vi "set Limit Line Setting.vi"(8 "error in (no error)":errorcluster, 9 "Turn On?":bool, 10 "Limit Line Setting":T1={"Limit Line Index"=1, "Frequency Table"=[], "Amplitude Table"=[], "Name"=""} {"Limit Line Index" min=1 max=8}, 11 "Keysight 9020A in":refnum<class "Keysight 9020A.lvclass">) -> (0 "error out":errorcluster, 3 "Keysight 9020A out":refnum<class "Keysight 9020A.lvclass">)   [LabVIEW 2023, in "Spectrum Analyzer.lvlib" / "Keysight 9020A.lvclass"]
uses:
  Keysight 9020A.lvclass
  TYPE DEFINITION/TYPE Limit Line Setting Table.ctl
  Keysight 9020A.lvclass/Keysight 9020A.ctl
  Spectrum Analyzer.lvlib
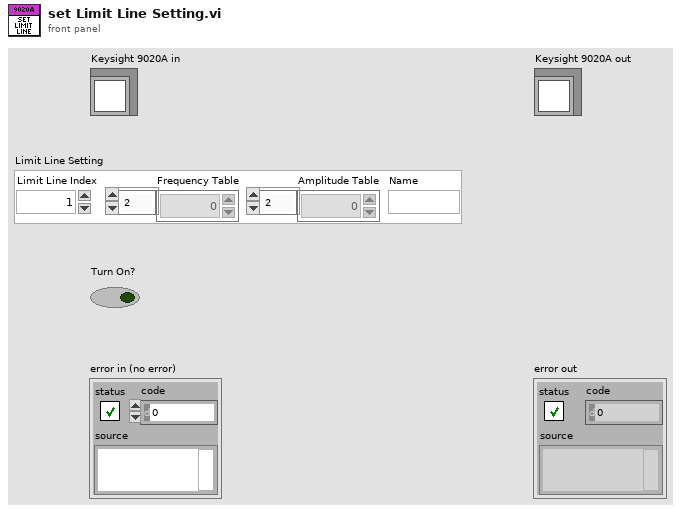
[diagram p1: front panel]
types:
  T1 = typedef "Spectrum Analyzer.lvlib/TYPE Limit Line Setting Table.ctl" = cluster{"Limit Line Index":i32, "Frequency Table":dbl[], "Amplitude Table":dbl[], "Name":string}
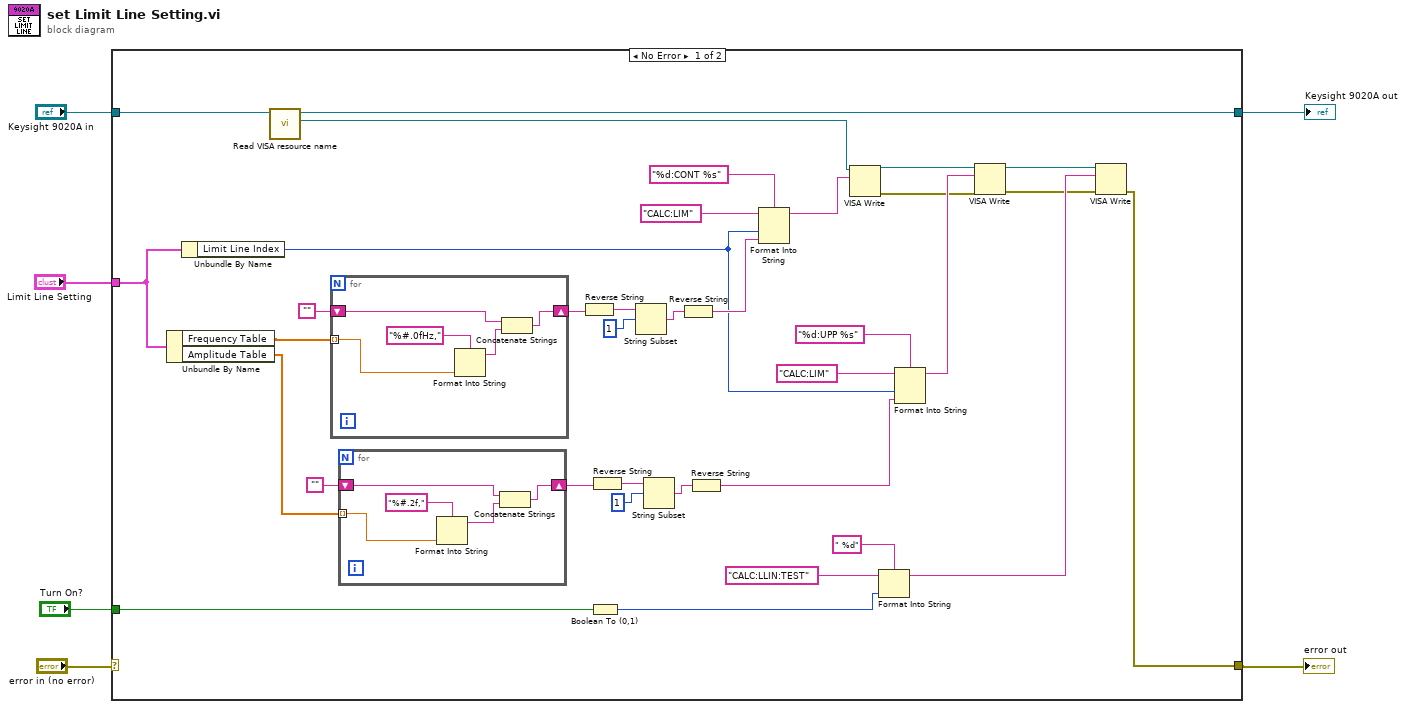
[diagram p0: block diagram]
diagram:
  n1 = case shown="No Error" "error in (no error)" {
    selector: "error in (no error)" -> [_ w52]
    tunnel: "Keysight 9020A in" -> [w40 w53]
    tunnel: [w41 w53] -> w5
    tunnel: [w8 w52] -> w3
    tunnel: "Limit Line Setting" -> [w33 _]
    tunnel: "Turn On?" -> [w15 _]
    frame No Error {
      n2 = Unbundle By Name(w33) -> ("Frequency Table"=w34:dbl[], "Amplitude Table"=w23:dbl[])
      n3 = Unbundle By Name(w33) -> ("Limit Line Index"=w20:i32)
      n4 = call "Read VISA resource name.vi"("Keysight 9020A in"=w40) -> ("VISA resource name"=w7:refnum<visa-resource-name>, "Keysight 9020A out"=w41:refnum<class "Keysight 9020A.lvclass">)  [unwired: 8 in, 1 out]
      n5 = for {
        tunnel: w34 -> [w47] mode=indexing
        shift-right: [w50] -> w38
        shift-left: "" -> [w51]
        n6 = Format Into String(format string="%#.0fHz,", w47) -> (resulting string=w48:string)  [unwired: 2 in, 1 out]
        n7 = Concatenate Strings(w51, w48) -> (w50:string)
      }
      n8 = for {
        tunnel: w23 -> [w44] mode=indexing
        shift-right: [w45] -> w25
        shift-left: "" -> [w46]
        n9 = Format Into String(format string="%#.2f,", w44) -> (resulting string=w43:string)  [unwired: 2 in, 1 out]
        n10 = Concatenate Strings(w46, w43) -> (w45:string)
      }
      n11 = Reverse String(1:w38) -> (0:w37:string)
      n12 = Boolean To (0,1)(Boolean=w15) -> (0, 1=w12:i16)
      n13 = Reverse String(1:w25) -> (0:w26:string)
      n14 = String Subset(string=w37, offset (0)=1) -> (substring=w35:string)  [unwired: 1 in]
      n15 = String Subset(string=w26, offset (0)=1) -> (substring=w28:string)  [unwired: 1 in]
      n16 = Reverse String(1:w35) -> (0:w30:string)
      n17 = Reverse String(1:w28) -> (0:w19:string)
      n18 = Format Into String(format string="%d:CONT %s", initial string="CALC:LIM", w20, w30) -> (resulting string=w29:string)  [unwired: 1 in, 1 out]
      n19 = VISA Write(VISA resource name=w7, write buffer=w29) -> (VISA resource name out=w18:refnum<visa-resource-name>, error out=w16:errorcluster)  [unwired: 1 in, 1 out]
      n20 = Format Into String(format string=" %d", initial string="CALC:LLIN:TEST", w12) -> (resulting string=w11:string)  [unwired: 1 in, 1 out]
      n21 = Format Into String(format string="%d:UPP %s", initial string="CALC:LIM", w20, w19) -> (resulting string=w17:string)  [unwired: 1 in, 1 out]
      n22 = VISA Write(VISA resource name=w18, write buffer=w17, error in (no error)=w16) -> (VISA resource name out=w10:refnum<visa-resource-name>, error out=w9:errorcluster)  [unwired: 1 out]
      n23 = VISA Write(VISA resource name=w10, write buffer=w11, error in (no error)=w9) -> (error out=w8:errorcluster)  [unwired: 2 out]
    }
    frame Error {
    }
  }
  "error out" <- w3
  "Keysight 9020A out" <- w5
